vi "DE10_control.vi"() -> ()   [LabVIEW 2014]
uses:
  <vilib>/Analysis/baseanly.llb/Mean (DBL).vi
  <vilib>/Utility/file.llb/Write To Spreadsheet File (I64).vi
  <vilib>/Analysis/NI_AALBase.lvlib
panel:
  in  "Update Ch gain cal":bool
  in  "Ch Gain Cal.":T1={"A:LG"=60, "A:MG"=60, "A:HG"=60, "B:LG"=60, "B:MG"=60, "B:HG"=60, "C:LG"=60, "C:MG"=60, "C:HG"=60, "D:LG"=60, "D:MG"=60, "D:HG"=60}
  out "Average":i32=10
  in  "read back":i32=1024
  out "Counter":u16=23
  in  "Update Act ch sel":bool
  in  "Active Channel":enum32{"Ch A", "Ch B", "Ch C", "Ch D"}(radio)
  in  "flash 2 buf":bool
  in  "Write to flash":bool
  in  "Load from flash":bool
  in  "Clear Graph":bool
  out "Avg_A (uA)":dbl(graph)
  out "Peak_A (uA)":dbl(graph)
  out "Avg_A (uA)":sgl=1024.0
  in  "AFE Gain Selection":enum32{"LG", "MG", "HG"}(radio)
  in  "Register Name":u16(ring) items=["BL:G1:A", "FFIFO:WD", "BL:LEN", "EVT:TAIL", "EVT:LEN", "TRIG:DL", "TRIG:DT", "TRIG:TH", "CR", "NF:SUM", "NF:DOSX", "NF:DOSY", "THRSH", "BL:G1:A", "BL:G2:A", "BL:G3:A", "CH:SEL", "OFFS:A", "OFFS:B", "OFFS:C", "OFFS:D", "TRIP:X:MAX", "TRIP:X:MIN", "TRIP:Y:MAX", "TRIP:Y:MIN", ""]
  in  "Value (Decimal)":i32
  out "STRING OUT":string
  out "DEC  OUT":i32
  out "HEX  OUT":i32 format="%x"
  in  "Register Name 2":u16(ring) items=["", "PEAK?", "FW?", "PW?", "TRIG:DL?", "CH:SEL?", "TRIG:TH?", "BL:G3:A?", "BL:G1:C?", "BL:G2:C?", "BL:G3:C?", "BL:G1:B?", "BL:G2:B?", "BL:G3:B?", "FIFO:WD?", "FFIFO:A?", "EVT:TAIL?", "SR?", "CR?", "NF:DOS?", "NF:SUM?", "THRSH?", "X:INST?", "Y:INST?", "S:INST?", "X:AVER?", "Y:AVER?", "S:AVER?", "S:RAW?", "BL:G1:A?", "BL:G2:A?", "BL:G3:A?", "GAIN:D?", "OFFS:A?", "OFFS:B?", "OFFS:C?", "OFFS:D?", "DEBUG:A?", "DEBUG:B?", "DEBUG:C?", "DEBUG:D?", "DEBUG:MOD?", "DEBUG:BUF:A?", "DEBUG:BUF:B?", "DEBUG:BUF:C?", "DEBUG:BUF:D?", "TRIG:MASK?", "AFE:CTRL?", "TRIP:X:MAX?", "TRIP:X:MIN?", "TRIP:Y:MAX?", "TRIP:Y:MIN?", "DATA:BUF:1?", "DATA:BUF:2?", "DATA:BUF:3?", "DATA:BUF:4?", "DATA:BUF:5?"]
  in  "ARBRwrite":bool
  in  "ARBRread":bool
  out "Duty cycle (%)":sgl=1024.0
  out "Freqquency (Hz)":i32=1024
  out "pulse width(us)":i16=1024
  out "Peak_A (uA)":sgl=1024.0
  in  "FIFO clear":bool
  in  "update to flash buf":bool
  in  "MAC":i32[](array[numeric]) format="%02x"
  in  "IP":i32[](array[numeric])
  out "MB Firmware ver:":string="FPGA_VER?"
  in  "Update Ch BL":bool
  in  "Ch BL Adj.":T2={"A:BL1"=60, "A:BL2"=60, "A:BL3"=60, "B:BL1"=60, "B:BL2"=60, "B:BL3"=60, "C:BL1"=60, "C:BL2"=60, "C:BL3"=60, "DBL1"=60, "D:BL2"=60, "D:BL3"=60}
  in  "Update AFE control reg":bool
  in  "Update  mode reg":bool
  in  "Mode Register":T3={"Run"=FALSE, "External Trigger"=TRUE, "Self Trigger"=TRUE, "Internal Trigger"=TRUE, "Trigger out enable"=TRUE, "Not in use"=TRUE, "BLR readout"=TRUE, "Bypass BLR"=TRUE, "AFE Cal"=FALSE, "Not in use"=FALSE}
  in  "Update Event Parameters":bool
  in  "Event Parameters":T4={"TRIG:TH"=1000, "TRIG:DT"=0, "TRIG:DL"=300, "EVT:LEN"=1024, "EVT:TAIL"=300, "OVERSHOOT\n< 256"=100}
  out "FPGA ver:":string="FPGA_VER?"
  out "Event data path:":path
  in  "Save data":bool
  in  "Log Evt data:":bool
  out "Fast FIFO Words":i32=4096
  in  "Event Data Log":bool
  out "ADC 16 bit data RAW or after BLR/Gain Cor.":i16[](graph)
  out "AFE Conl REGISTER":bool[](array[boolean])
  out "MODE REGISTER":bool[](array[boolean])
  out "STATUS REGISTER":bool[](array[boolean])
  out "ERROR  REGISTER":bool[](array[boolean])
  out "error out":errorcluster
  in  "stop":bool
  in  "IP ADRESS":string="192.168.12.10"
  # "History:  Oct 26.2017, Jan29,2018, May29,2018,Aug21,2018\nCal: 10 uA -> 1600 @ G= 100, so I = ADC*10/(16*G)\nChannel Gain Cal: 1 ~ 511, = 1/256 ~ 511/256, so 256 is no adjust."
  # "ELinac Faraday Cup Data Acquisition/Control  Rev 1.0, SL, Oct. 26 2017"
  # "0     1     2     3     4     5     6    7      8     9    10   11   12   13    14  15"
  # "A0  A1"
  # "0     1     2     3     4     5     6    7      8     9    10   11   12   13    14  15"
  # "Run"
  # "0     1     2     3     4     5     6    7      8     9    10   11   12   13    14  15"
  # "0     1     2     3     4     5     6    7      8     9    10   11   12   13    14  15"
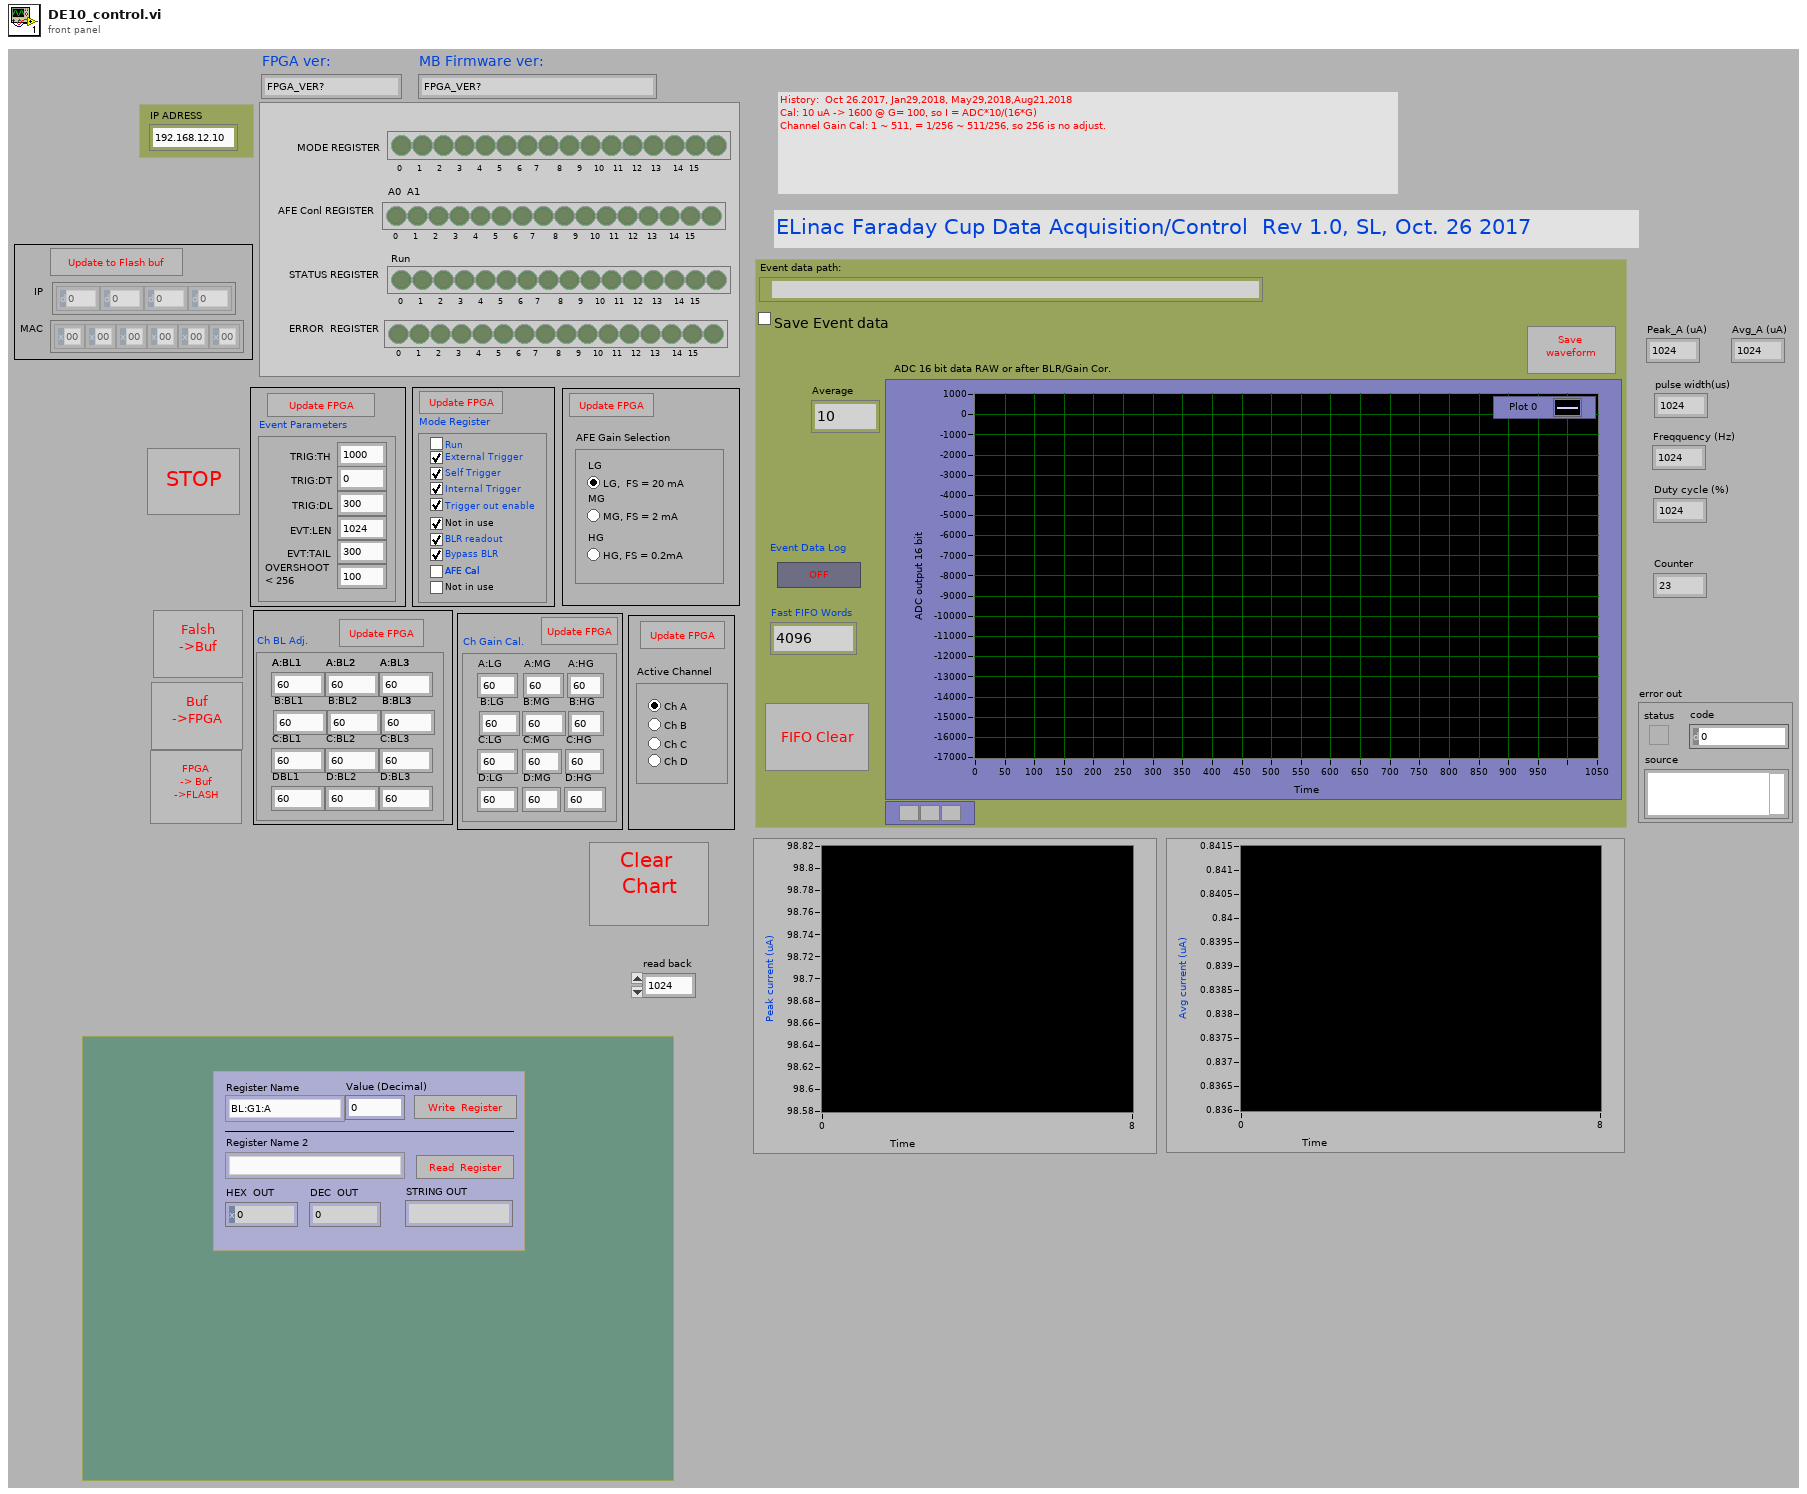
[diagram p1: front panel]
types:
  T1 = cluster{"A:LG":i16, "A:MG":i16, "A:HG":i16, "B:LG":i16, "B:MG":i16, "B:HG":i16, "C:LG":i16, "C:MG":i16, "C:HG":i16, "D:LG":i16, "D:MG":i16, "D:HG":i16}
  T2 = cluster{"A:BL1":i16, "A:BL2":i16, "A:BL3":i16, "B:BL1":i16, "B:BL2":i16, "B:BL3":i16, "C:BL1":i16, "C:BL2":i16, "C:BL3":i16, "DBL1":i16, "D:BL2":i16, "D:BL3":i16}
  T3 = cluster{"Run":bool, "External Trigger":bool, "Self Trigger":bool, "Internal Trigger":bool, "Trigger out enable":bool, "Not in use":bool, "BLR readout":bool, "Bypass BLR":bool, "AFE Cal":bool, "Not in use":bool}
  T4 = cluster{"TRIG:TH":u16, "TRIG:DT":u16, "TRIG:DL":u16, "EVT:LEN":u16, "EVT:TAIL":u16, "OVERSHOOT\n< 256":u16}
  T5 = cluster{bool, bool, bool, bool, bool, bool, bool, bool, bool, bool}
  T6 = cluster{"number out":i32, "number out":i32, "number out":i32, "number out":i32, "number out":i32, "number out":i32}
  T7 = cluster{"number out":i32, "number out":i32, "number out":i32, "number out":i32, "number out":i32, "number out":i32, "number out":i32, "number out":i32, "number out":i32, "number out":i32, "number out":i32, "number out":i32}
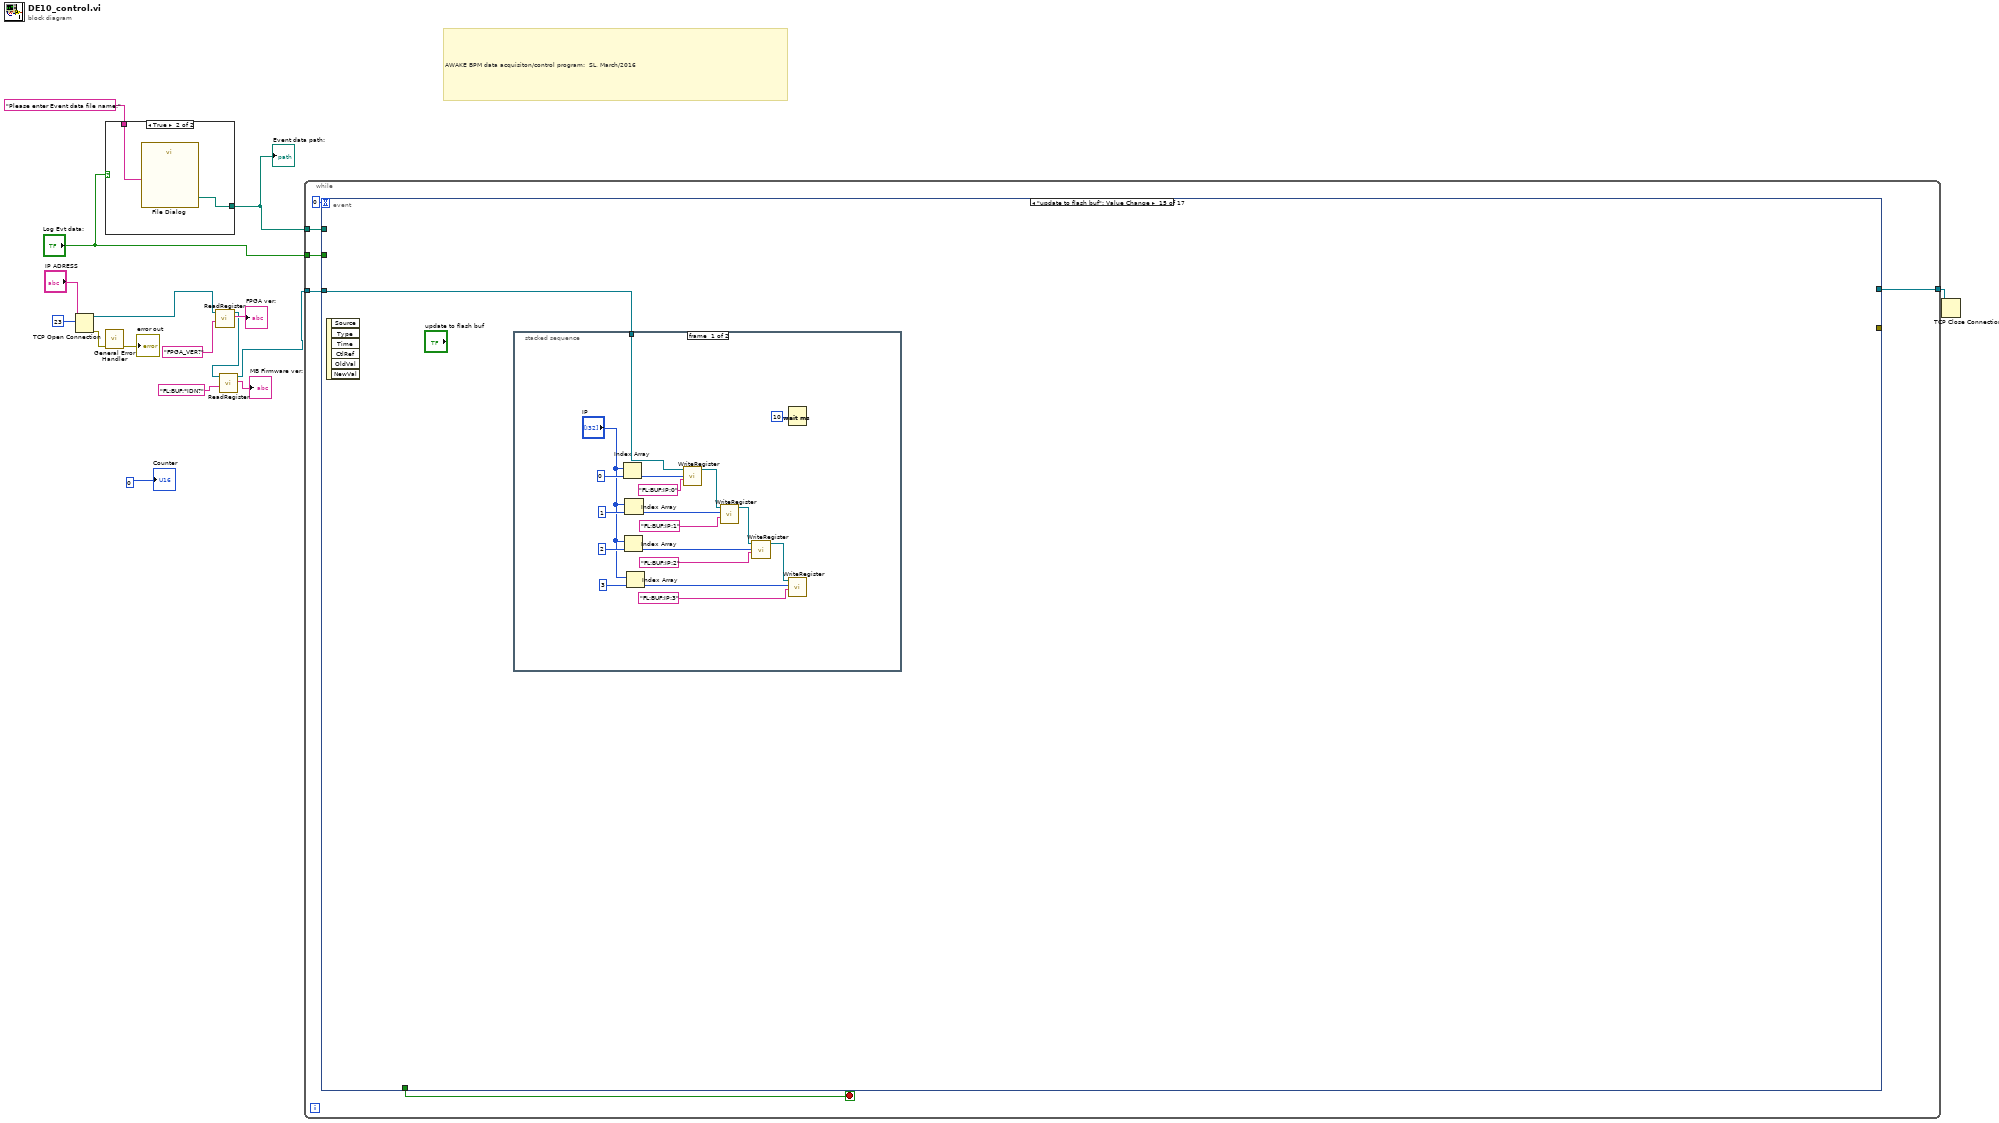
[diagram p0: block diagram]
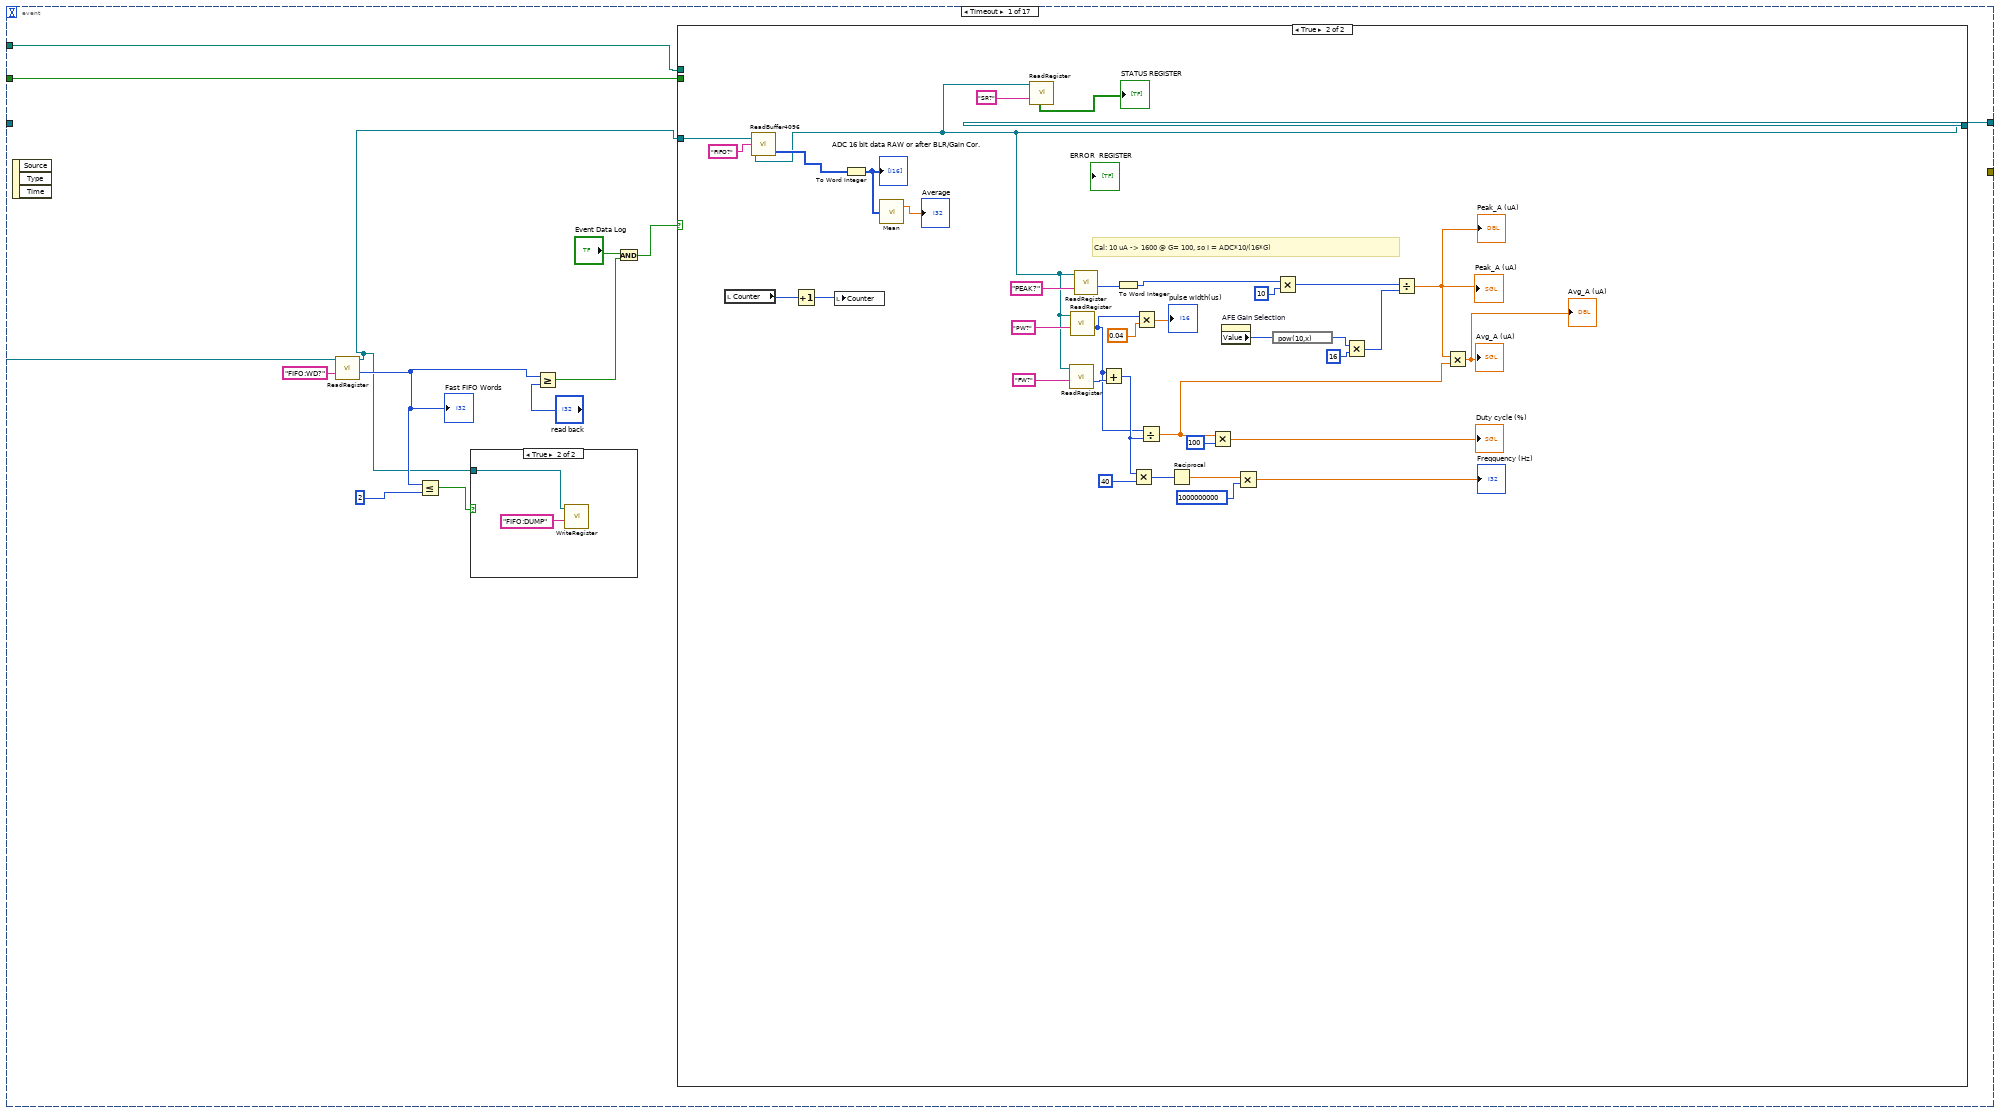
[diagram p3: hidden frame]
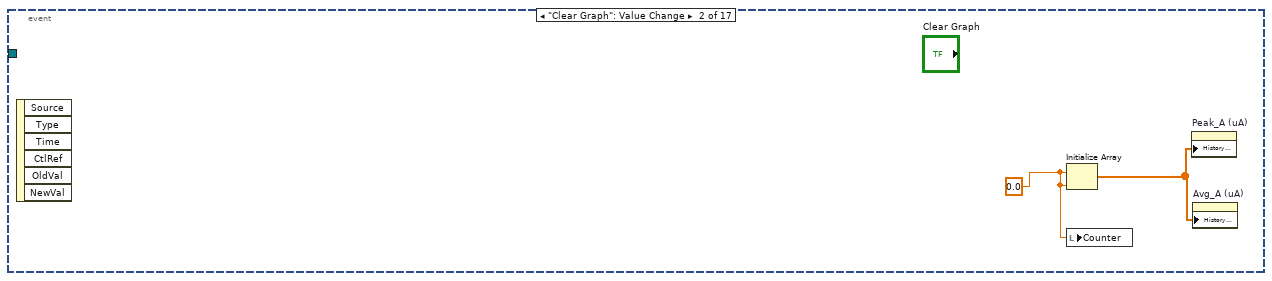
[diagram p6: hidden frame]
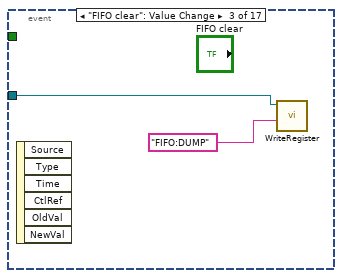
[diagram p7: hidden frame]
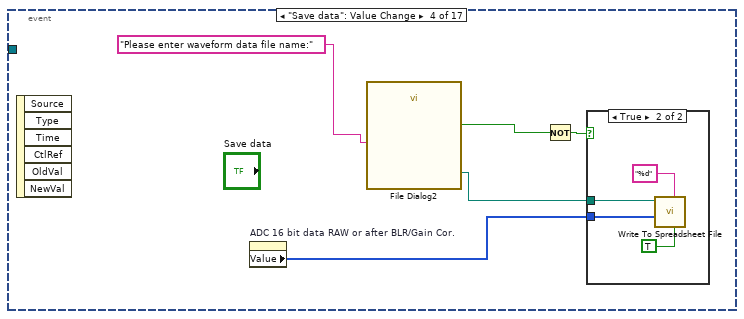
[diagram p8: hidden frame]
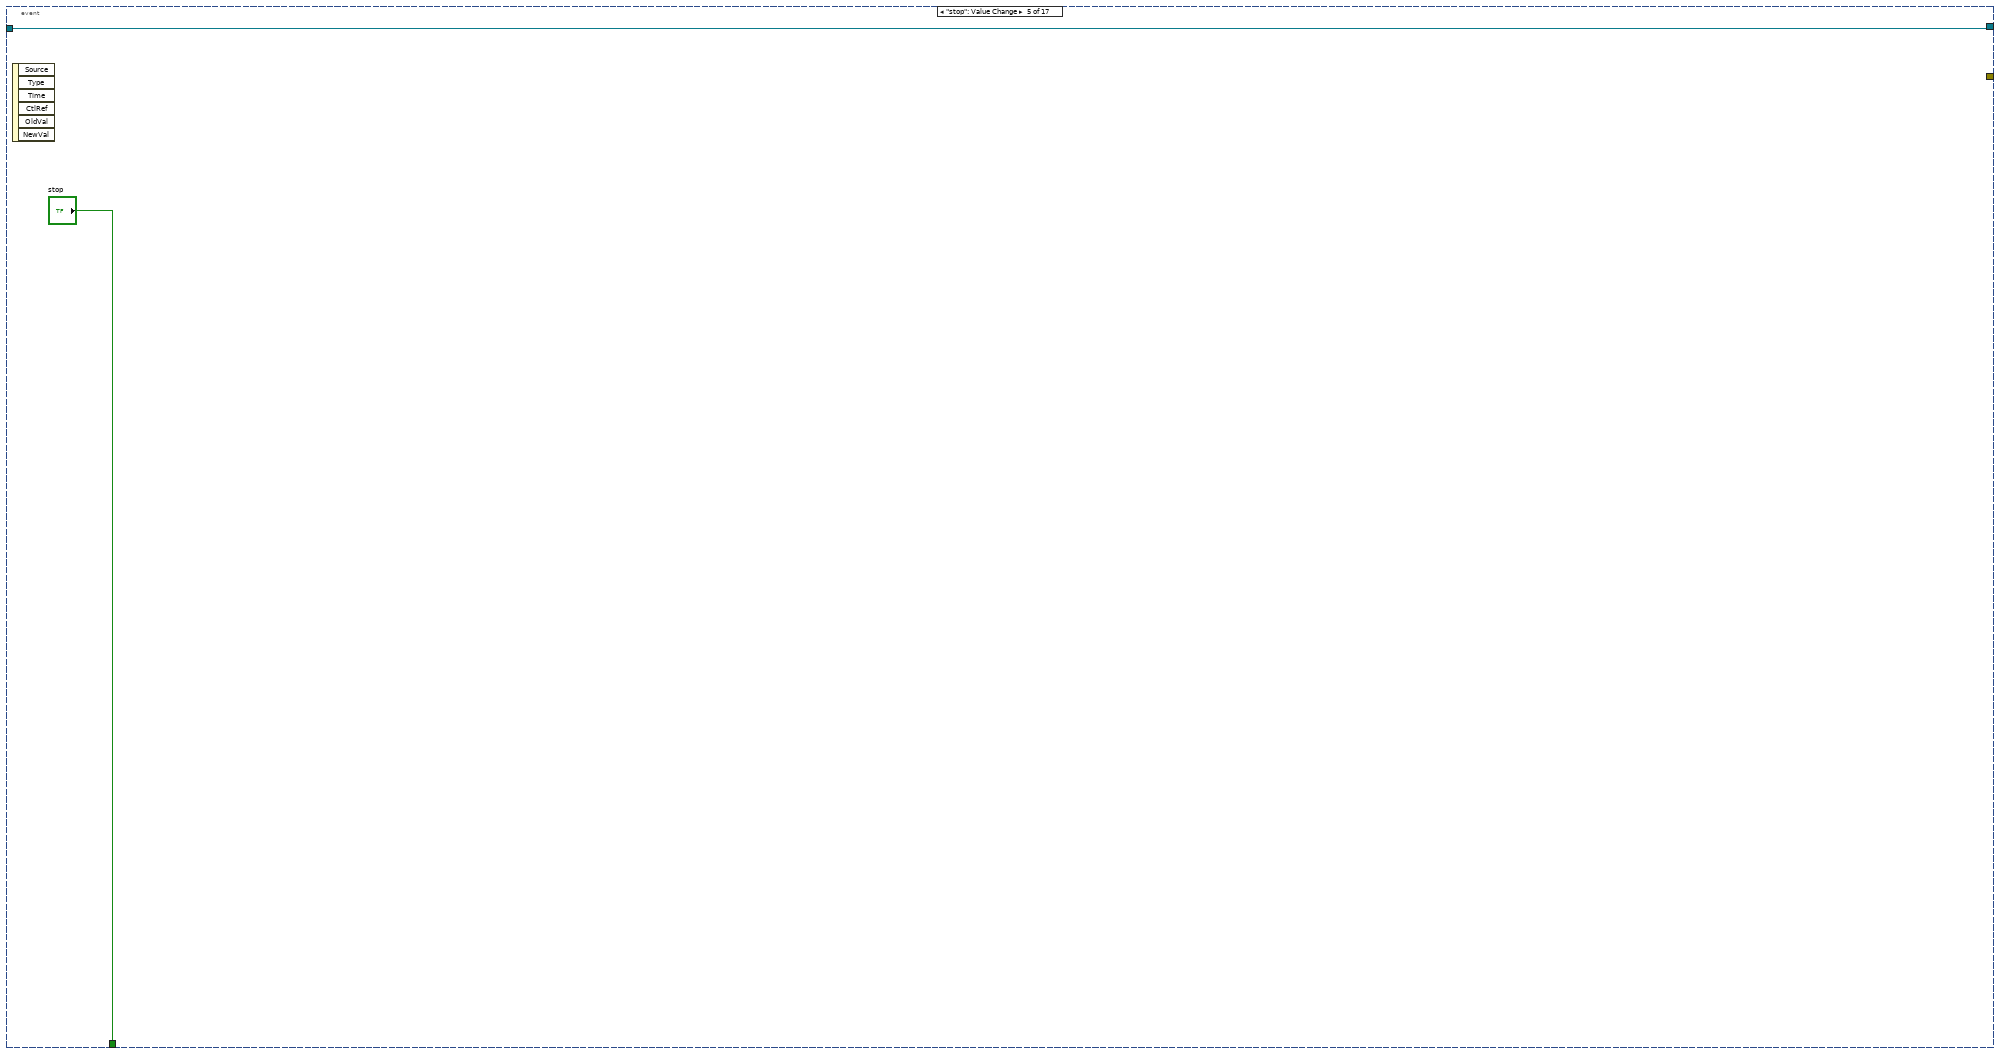
[diagram p10: hidden frame]
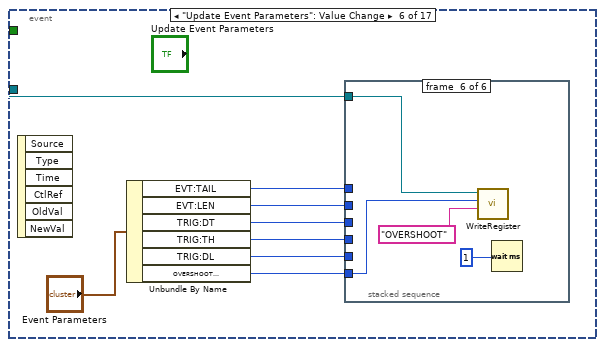
[diagram p11: hidden frame]
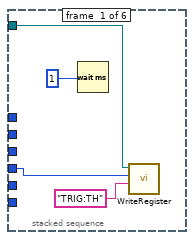
[diagram p12: hidden frame]
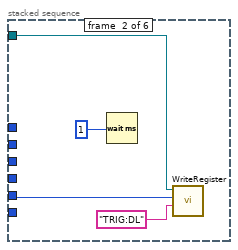
[diagram p13: hidden frame]
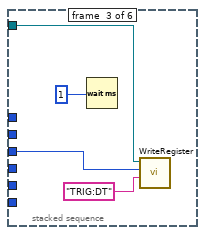
[diagram p14: hidden frame]
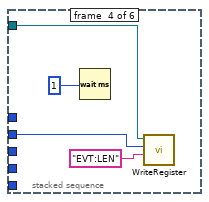
[diagram p15: hidden frame]
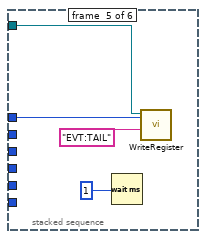
[diagram p16: hidden frame]
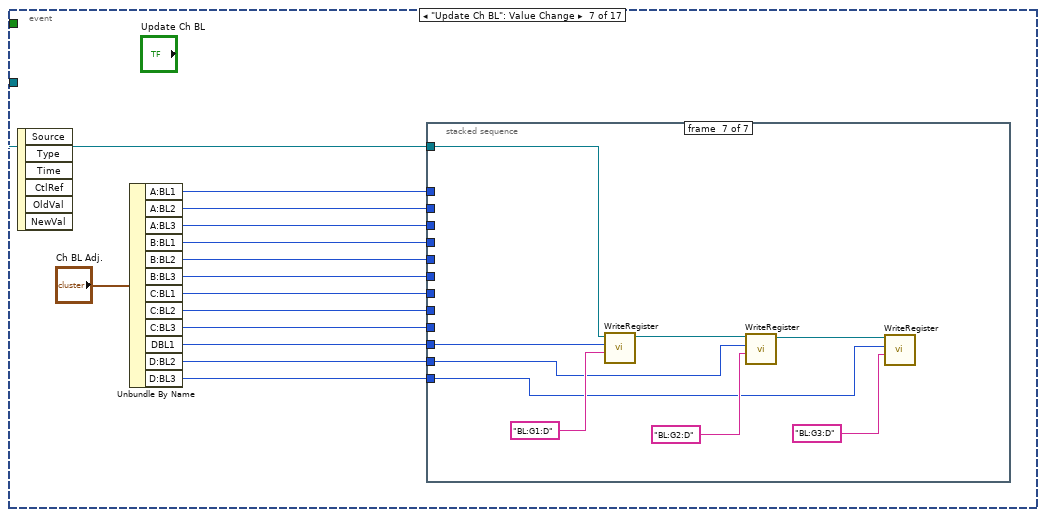
[diagram p17: hidden frame]
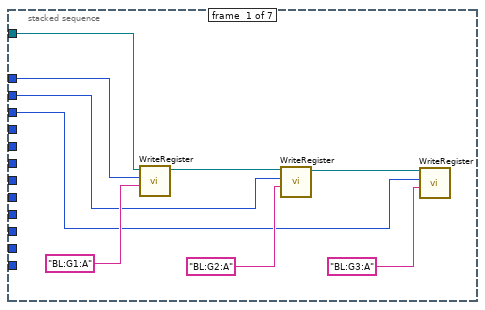
[diagram p18: hidden frame]
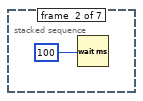
[diagram p19: hidden frame]
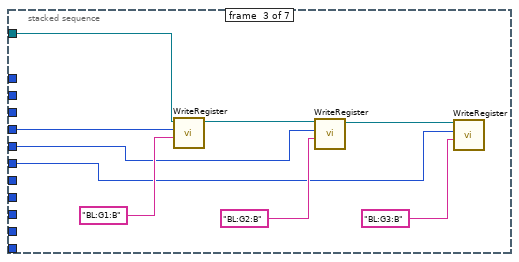
[diagram p20: hidden frame]
diagram:
  # "AWAKE BPM data acquisiton/control program:  SL, March/2016"
  n1 = TCP Open Connection(address="IP ADRESS", remote port or service name=u16 23 ("REMOTE PORT")) -> (connection ID=w8:refnum<k5>, error out=w14:errorcluster)  [unwired: 3 in]
  n2 = call <vilib>:"General Error Handler.vi"("error in (no error)"=w14) -> ("error out"=→"error out":errorcluster)  [unwired: 10 in, 4 out]
  n3 = case shown="True" "Log Evt data:" {
    tunnel: [_ w18] -> w9
    tunnel: "Please enter Event data file name:" -> [_ w17]
    frame False {
    }
    frame True {
      n4 = call "File Dialog"("prompt"=w17) -> ("selected path"=w18:path)  [unwired: 11 in, 3 out]
    }
  }
  "Event data path:" <- w9
  n5 = call "ReadRegister.vi"("string in"="FPGA_VER?", "connection ID in"=w8) -> ("string out"=→"FPGA ver:":string, "connection ID out"=w3:refnum<k5>)  [unwired: 3 in, 3 out]
  n6 = call "ReadRegister.vi"("string in"="FL:BUF:*IDN?", "connection ID in"=w3) -> ("string out"=→"MB Firmware ver:":string, "connection ID out"=w2:refnum<k5>)  [unwired: 3 in, 3 out]
  n7 = while {
    tunnel: w2 -> [w23]
    tunnel: [w22] -> w12
    tunnel: "Log Evt data:" -> [w20]
    tunnel: w9 -> [w19]
    stop <- w24 stop-if-true
    n8 = event shown="[14] \"update to flash buf\": Value Change" {
      selector: _ -> [_ _ _ _ _ _ _ _ _ _ _ _ _ _ _ _ _]
      dyn-events: _ -> [_ _ _ _ _ _ _ _ _ _ _ _ _ _ _ _ _]
      timeout: 0 -> [_ _ _ _ _ _ _ _ _ _ _ _ _ _ _ _ _]
      tunnel: [_ _ _ _ "stop" _ _ _ _ _ _ _ _ _ _ _ _] -> w24
      tunnel: w23 -> [w35 _ w79 _ w90 w94 w136 w177 w230 w233 w260 w262 w270 w416 w421 w468 w485]
      tunnel: [w36 _ _ _ w90 _ _ _ _ _ w257 _ _ _ _ _ w482] -> w22
      tunnel: [_ _ _ _ _ _ _ _ _ _ w253 _ _ _ _ _ w478] -> _
      tunnel: w20 -> [w33 _ _ _ _ _ _ _ _ _ _ _ _ _ _ _ _]
      tunnel: w19 -> [w32 _ _ _ _ _ _ _ _ _ _ _ _ _ _ _ _]
      event Timeout {
        n9 = event-data() -> ()  [unwired: 1 in, 3 out]
        n10 = call "ReadRegister.vi"("string in"="FIFO:WD?", "connection ID in"=w35) -> ("number out"=w27:i32, "connection ID out"=w25:refnum<k5>)  [unwired: 3 in, 3 out]
        "Fast FIFO Words" <- w27
        n11 = Less Or Equal?(x=w27, y=2) -> (x <= y?=w26:bool)
        n12 = case shown="True" w26 {
          tunnel: w25 -> [_ w38]
          frame False {
          }
          frame True {
            n13 = call "WriteRegister.vi"("string in"="FIFO:DUMP", "connection ID in"=w38) -> ()  [unwired: 6 in, 2 out]
          }
        }
        n14 = Greater Or Equal?(x=w27, y="read back") -> (x >= y?=w30:bool)
        n15 = And(x="Event Data Log", y=w30) -> (x .and. y?=w37:bool)
        n16 = case shown="True" w37 {
          tunnel: [w40 w46] -> w36
          tunnel: w25 -> [w40 w76]
          tunnel: w33 -> [_ _]
          tunnel: w32 -> [_ _]
          frame False {
          }
          frame True {
            # "Cal: 10 uA -> 1600 @ G= 100, so I = ADC*10/(16*G)"
            n17 = local read "Counter"() -> (w44:u16)
            n18 = call "ReadBuffer4096.vi"("string in"="FIFO?", "connection ID in"=w76) -> ("FIFO32_data"=w49:u32[], "connection ID out"=w46:refnum<k5>)  [unwired: 2 in]
            n19 = Increment(x=w44) -> (x+1=w43:u16)
            n20 = local write "Counter"(w43) -> ()
            n21 = To Word Integer(number=w49) -> (16bit integer=w42:i16[])
            "ADC 16 bit data RAW or after BLR/Gain Cor." <- w42
            n22 = call-poly <vilib>:"Mean.vi"("X"=w42) -> ("mean"=→"Average":dbl)  [unwired: 1 out]
            n23 = call "ReadRegister.vi"("string in"="SR?", "connection ID in"=w46) -> ("boolean array out"=→"STATUS REGISTER":bool[])  [unwired: 3 in, 4 out]
            n24 = call "ReadRegister.vi"("string in"="FW?", "connection ID in"=w46) -> ("number out"=w72:i32)  [unwired: 3 in, 4 out]
            n25 = call "ReadRegister.vi"("string in"="PW?", "connection ID in"=w46) -> ("number out"=w66:i32)  [unwired: 3 in, 4 out]
            n26 = call "ReadRegister.vi"("string in"="PEAK?", "connection ID in"=w46) -> ("number out"=w59:i32)  [unwired: 3 in, 4 out]
            n27 = Add(x=w66, y=w72) -> (x+y=w69:i32)
            n28 = To Word Integer(number=w59) -> (16bit integer=w58:i16)
            n29 = Multiply(x=w69, y=40) -> (x*y=w70:i32)
            n30 = Multiply(x=w66, y=0.04) -> (x*y=→"pulse width(us)":dbl)
            n31 = Divide(x=w66, y=w69) -> (x/y=w52:dbl)
            n32 = Reciprocal(x=w70) -> (1/x=w64:dbl)
            n33 = Multiply(x=w52, y=100) -> (x*y=→"Duty cycle (%)":dbl)
            n34 = property on="AFE Gain Selection" class="RadioBtnsControl (strict)"() -> ("Value"=w55:enum32{"LG", "MG", "HG"})  [unwired: 2 in, 2 out]
            n35 = Multiply(x=w64, y=1000000000) -> (x*y=→"Freqquency (Hz)":dbl)
            n36 = expression code="pow(10,x)"(w55) -> (w56:enum32{"LG", "MG", "HG"})
            n37 = Multiply(x=w58, y=10) -> (x*y=w60:i32)
            n38 = Multiply(x=w56, y=16) -> (x*y=w54:u32)
            n39 = Divide(x=w60, y=w54) -> (x/y=w51:dbl)
            "Peak_A (uA)" <- w51
            "Peak_A (uA)" <- w51
            n40 = Multiply(x=w51, y=w52) -> (x*y=→"Avg_A (uA)" →"Avg_A (uA)":dbl)
          }
        }
      }
      event "Clear Graph": Value Change {
        w77 = sgl 0.0
        n41 = event-data() -> ()  [unwired: 1 in, 6 out]
        n42 = Initialize Array(w77, w77) -> (w78:sgl[])
        n43 = local write "Counter"(w77) -> ()
        n44 = property on="Peak_A (uA)" class="WFChart (strict)"("History Data"=w78) -> ()  [unwired: 2 in, 2 out]
        n45 = property on="Avg_A (uA)" class="WFChart (strict)"("History Data"=w78) -> ()  [unwired: 2 in, 2 out]
      }
      event "FIFO clear": Value Change {
        n46 = event-data() -> ()  [unwired: 1 in, 6 out]
        n47 = call "WriteRegister.vi"("string in"="FIFO:DUMP", "connection ID in"=w79) -> ()  [unwired: 6 in, 2 out]
      }
      event "Save data": Value Change {
        n48 = event-data() -> ()  [unwired: 1 in, 6 out]
        n49 = property on="ADC 16 bit data RAW or after BLR/Gain Cor." class="WFGraph (strict)"() -> ("Value"=w82:i16[])  [unwired: 2 in, 2 out]
        n50 = call "File Dialog2"("prompt"="Please enter waveform data file name:") -> ("selected path"=w81:path, "cancelled"=w83:bool)  [unwired: 11 in, 2 out]
        n51 = Not(x=w83) -> (.not. x?=w84:bool)
        n52 = case shown="True" w84 {
          tunnel: w82 -> [_ w86]
          tunnel: w81 -> [_ w87]
          frame False {
          }
          frame True {
            n53 = call-poly <vilib>:"Write To Spreadsheet File.vi"("transpose? (no:F)"=TRUE, "format (%d)"="%d", "1D data"=w86, "file path (dialog if empty)"=w87) -> ()  [unwired: 4 in, 1 out]
          }
        }
      }
      event "stop": Value Change {
        n54 = event-data() -> ()  [unwired: 1 in, 6 out]
      }
      event "Update Event Parameters": Value Change {
        n55 = event-data() -> ()  [unwired: 1 in, 6 out]
        n56 = Unbundle By Name("Event Parameters") -> ("EVT:TAIL"=w98:u16, "EVT:LEN"=w93:u16, "TRIG:DT"=w97:u16, "TRIG:TH"=w96:u16, "TRIG:DL"=w95:u16, "OVERSHOOT\n< 256"=w92:u16)
        n57 = stacked-sequence {
          tunnel: w98 -> [_ _ _ _ w117 _]
          tunnel: w93 -> [_ _ _ w113 _ _]
          tunnel: w97 -> [_ _ w109 _ _ _]
          tunnel: w96 -> [w101 _ _ _ _ _]
          tunnel: w95 -> [_ w104 _ _ _ _]
          tunnel: w94 -> [w100 w105 w108 w112 w116 w122]
          tunnel: w92 -> [_ _ _ _ _ w121]
          frame #0 {
            n58 = Wait (ms)(milliseconds to wait=1 ("Value")) -> ()  [unwired: 1 out]
            n59 = call "WriteRegister.vi"("string in"="TRIG:TH", "value in"=w101, "connection ID in"=w100) -> ()  [unwired: 5 in, 2 out]
          }
          frame #1 {
            n60 = Wait (ms)(milliseconds to wait=1 ("Value")) -> ()  [unwired: 1 out]
            n61 = call "WriteRegister.vi"("string in"="TRIG:DL", "value in"=w104, "connection ID in"=w105) -> ()  [unwired: 5 in, 2 out]
          }
          frame #2 {
            n62 = Wait (ms)(milliseconds to wait=1 ("Value")) -> ()  [unwired: 1 out]
            n63 = call "WriteRegister.vi"("string in"="TRIG:DT", "value in"=w109, "connection ID in"=w108) -> ()  [unwired: 5 in, 2 out]
          }
          frame #3 {
            n64 = Wait (ms)(milliseconds to wait=1 ("Value")) -> ()  [unwired: 1 out]
            n65 = call "WriteRegister.vi"("string in"="EVT:LEN", "value in"=w113, "connection ID in"=w112) -> ()  [unwired: 5 in, 2 out]
          }
          frame #4 {
            n66 = Wait (ms)(milliseconds to wait=1 ("Value")) -> ()  [unwired: 1 out]
            n67 = call "WriteRegister.vi"("string in"="EVT:TAIL", "value in"=w117, "connection ID in"=w116) -> ()  [unwired: 5 in, 2 out]
          }
          frame #5 {
            n68 = call "WriteRegister.vi"("string in"="OVERSHOOT", "value in"=w121, "connection ID in"=w122) -> ()  [unwired: 5 in, 2 out]
            n69 = Wait (ms)(milliseconds to wait=1 ("Value")) -> ()  [unwired: 1 out]
          }
        }
      }
      event "Update Ch BL": Value Change {
        n70 = event-data() -> ()  [unwired: 1 in, 6 out]
        n71 = Unbundle By Name("Ch BL Adj.") -> ("A:BL1"=w135:i16, "A:BL2"=w134:i16, "A:BL3"=w133:i16, "B:BL1"=w132:i16, "B:BL2"=w131:i16, "B:BL3"=w130:i16, "C:BL1"=w129:i16, "C:BL2"=w128:i16, "C:BL3"=w127:i16, "DBL1"=w126:i16, "D:BL2"=w125:i16, "D:BL3"=w124:i16)
        n72 = stacked-sequence {
          tunnel: w136 -> [w145 _ w151 _ w161 _ w171]
          tunnel: w135 -> [w144 _ _ _ _ _ _]
          tunnel: w134 -> [w139 _ _ _ _ _ _]
          tunnel: w133 -> [w138 _ _ _ _ _ _]
          tunnel: w132 -> [_ _ w150 _ _ _ _]
          tunnel: w131 -> [_ _ w149 _ _ _ _]
          tunnel: w130 -> [_ _ w148 _ _ _ _]
          tunnel: w129 -> [_ _ _ _ w160 _ _]
          tunnel: w128 -> [_ _ _ _ w159 _ _]
          tunnel: w127 -> [_ _ _ _ w158 _ _]
          tunnel: w126 -> [_ _ _ _ _ _ w170]
          tunnel: w125 -> [_ _ _ _ _ _ w169]
          tunnel: w124 -> [_ _ _ _ _ _ w168]
          frame #0 {
            n73 = call "WriteRegister.vi"("string in"="BL:G1:A", "value in"=w144, "connection ID in"=w145) -> ("connection ID out"=w141:refnum<k5>)  [unwired: 5 in, 1 out]
            n74 = call "WriteRegister.vi"("string in"="BL:G2:A", "value in"=w139, "connection ID in"=w141) -> ("connection ID out"=w140:refnum<k5>)  [unwired: 5 in, 1 out]
            n75 = call "WriteRegister.vi"("string in"="BL:G3:A", "value in"=w138, "connection ID in"=w140) -> ()  [unwired: 5 in, 2 out]
          }
          frame #1 {
            n76 = Wait (ms)(milliseconds to wait=100 ("Value")) -> ()  [unwired: 1 out]
          }
          frame #2 {
            n77 = call "WriteRegister.vi"("string in"="BL:G1:B", "value in"=w150, "connection ID in"=w151) -> ("connection ID out"=w153:refnum<k5>)  [unwired: 5 in, 1 out]
            n78 = call "WriteRegister.vi"("string in"="BL:G2:B", "value in"=w149, "connection ID in"=w153) -> ("connection ID out"=w152:refnum<k5>)  [unwired: 5 in, 1 out]
            n79 = call "WriteRegister.vi"("string in"="BL:G3:B", "value in"=w148, "connection ID in"=w152) -> ()  [unwired: 5 in, 2 out]
          }
          frame #3 {
            n80 = Wait (ms)(milliseconds to wait=100 ("Value")) -> ()  [unwired: 1 out]
          }
          frame #4 {
            n81 = call "WriteRegister.vi"("string in"="BL:G1:C", "value in"=w160, "connection ID in"=w161) -> ("connection ID out"=w163:refnum<k5>)  [unwired: 5 in, 1 out]
            n82 = call "WriteRegister.vi"("string in"="BL:G2:C", "value in"=w159, "connection ID in"=w163) -> ("connection ID out"=w162:refnum<k5>)  [unwired: 5 in, 1 out]
            n83 = call "WriteRegister.vi"("string in"="BL:G3:C", "value in"=w158, "connection ID in"=w162) -> ()  [unwired: 5 in, 2 out]
          }
          frame #5 {
            n84 = Wait (ms)(milliseconds to wait=100 ("Value")) -> ()  [unwired: 1 out]
          }
          frame #6 {
            n85 = call "WriteRegister.vi"("string in"="BL:G1:D", "value in"=w170, "connection ID in"=w171) -> ("connection ID out"=w173:refnum<k5>)  [unwired: 5 in, 1 out]
            n86 = call "WriteRegister.vi"("string in"="BL:G2:D", "value in"=w169, "connection ID in"=w173) -> ("connection ID out"=w172:refnum<k5>)  [unwired: 5 in, 1 out]
            n87 = call "WriteRegister.vi"("string in"="BL:G3:D", "value in"=w168, "connection ID in"=w172) -> ()  [unwired: 5 in, 2 out]
          }
        }
      }
      event "Update Ch gain cal": Value Change {
        n88 = event-data() -> ()  [unwired: 1 in, 6 out]
        n89 = Unbundle By Name("Ch Gain Cal.") -> ("A:LG"=w189:i16, "A:MG"=w188:i16, "A:HG"=w187:i16, "B:LG"=w186:i16, "B:MG"=w185:i16, "B:HG"=w184:i16, "C:LG"=w183:i16, "C:MG"=w182:i16, "C:HG"=w181:i16, "D:LG"=w180:i16, "D:MG"=w179:i16, "D:HG"=w178:i16)
        n90 = stacked-sequence {
          tunnel: w177 -> [w198 _ w204 _ w214 _ w224]
          tunnel: w189 -> [w197 _ _ _ _ _ _]
          tunnel: w188 -> [w192 _ _ _ _ _ _]
          tunnel: w187 -> [w191 _ _ _ _ _ _]
          tunnel: w186 -> [_ _ w203 _ _ _ _]
          tunnel: w185 -> [_ _ w202 _ _ _ _]
          tunnel: w184 -> [_ _ w201 _ _ _ _]
          tunnel: w183 -> [_ _ _ _ w213 _ _]
          tunnel: w182 -> [_ _ _ _ w212 _ _]
          tunnel: w181 -> [_ _ _ _ w211 _ _]
          tunnel: w180 -> [_ _ _ _ _ _ w223]
          tunnel: w179 -> [_ _ _ _ _ _ w222]
          tunnel: w178 -> [_ _ _ _ _ _ w221]
          frame #0 {
            n91 = call "WriteRegister.vi"("string in"="CAL:G1:A", "value in"=w197, "connection ID in"=w198) -> ("connection ID out"=w194:refnum<k5>)  [unwired: 5 in, 1 out]
            n92 = call "WriteRegister.vi"("string in"="CAL:G2:A", "value in"=w192, "connection ID in"=w194) -> ("connection ID out"=w193:refnum<k5>)  [unwired: 5 in, 1 out]
            n93 = call "WriteRegister.vi"("string in"="CAL:G3:A", "value in"=w191, "connection ID in"=w193) -> ()  [unwired: 5 in, 2 out]
          }
          frame #1 {
            n94 = Wait (ms)(milliseconds to wait=100 ("Value")) -> ()  [unwired: 1 out]
          }
          frame #2 {
            n95 = call "WriteRegister.vi"("string in"="CAL:G1:B", "value in"=w203, "connection ID in"=w204) -> ("connection ID out"=w206:refnum<k5>)  [unwired: 5 in, 1 out]
            n96 = call "WriteRegister.vi"("string in"="CAL:G2:B", "value in"=w202, "connection ID in"=w206) -> ("connection ID out"=w205:refnum<k5>)  [unwired: 5 in, 1 out]
            n97 = call "WriteRegister.vi"("string in"="CAL:G3:B", "value in"=w201, "connection ID in"=w205) -> ()  [unwired: 5 in, 2 out]
          }
          frame #3 {
            n98 = Wait (ms)(milliseconds to wait=100 ("Value")) -> ()  [unwired: 1 out]
          }
          frame #4 {
            n99 = call "WriteRegister.vi"("string in"="CAL:G1:C", "value in"=w213, "connection ID in"=w214) -> ("connection ID out"=w216:refnum<k5>)  [unwired: 5 in, 1 out]
            n100 = call "WriteRegister.vi"("string in"="CAL:G2:C", "value in"=w212, "connection ID in"=w216) -> ("connection ID out"=w215:refnum<k5>)  [unwired: 5 in, 1 out]
            n101 = call "WriteRegister.vi"("string in"="CAL:G3:C", "value in"=w211, "connection ID in"=w215) -> ()  [unwired: 5 in, 2 out]
          }
          frame #5 {
            n102 = Wait (ms)(milliseconds to wait=100 ("Value")) -> ()  [unwired: 1 out]
          }
          frame #6 {
            n103 = call "WriteRegister.vi"("string in"="CAL:G1:D", "value in"=w223, "connection ID in"=w224) -> ("connection ID out"=w226:refnum<k5>)  [unwired: 5 in, 1 out]
            n104 = call "WriteRegister.vi"("string in"="CAL:G2:D", "value in"=w222, "connection ID in"=w226) -> ("connection ID out"=w225:refnum<k5>)  [unwired: 5 in, 1 out]
            n105 = call "WriteRegister.vi"("string in"="CAL:G3:D", "value in"=w221, "connection ID in"=w225) -> ()  [unwired: 5 in, 2 out]
          }
        }
      }
      event "ARBRwrite": Value Change {
        n106 = event-data() -> ()  [unwired: 1 in, 6 out]
        n107 = property on="Register Name" class="Ring (strict)"() -> ("RingText.Text"=w232:string)  [unwired: 2 in, 2 out]
        n108 = call "WriteRegister.vi"("string in"=w232, "value in"="Value (Decimal)", "connection ID in"=w230) -> ()  [unwired: 5 in, 2 out]
      }
      event "ARBRread": Value Change {
        n109 = event-data() -> ()  [unwired: 1 in, 6 out]
        n110 = property on="Register Name 2" class="Ring (strict)"() -> ("RingText.Text"=w236:string)  [unwired: 2 in, 2 out]
        n111 = call "ReadRegister.vi"("string in"=w236, "connection ID in"=w233) -> ("number out"=→"HEX  OUT" →"DEC  OUT":i32, "string out"=→"STRING OUT":string)  [unwired: 3 in, 3 out]
      }
      event "Update  mode reg": Value Change {
        w246 = FALSE
        n112 = event-data() -> ()  [unwired: 1 in, 6 out]
        n113 = Unbundle By Name("Mode Register") -> ("Run"=w251:bool, "Bypass BLR"=w247:bool, "BLR readout"=w248:bool, "Trigger out enable"=w239:bool, "Not in use"=w249:bool, "AFE Cal"=w250:bool, "Self Trigger"=w244:bool, "Internal Trigger"=w241:bool, "External Trigger"=w245:bool, "Not in use"=w238:bool)
        n114 = Not(x=w245) -> (.not. x?=w242:bool)
        n115 = And(x=w244, y=w242) -> (x .and. y?=w243:bool)
        n116 = And(x=w241, y=w242) -> (x .and. y?=w240:bool)
        n117 = Build Array(w251, w243, w240, w239, w239, w238, w246, w246, w248, w247, w246, w246, w246, w250, w249, w246) -> (w261:bool[])
        n118 = Boolean Array To Number(Boolean array=w261) -> (number=w237:u32)
        n119 = call "WriteRegister.vi"("string in"="CR", "value in"=w237, "connection ID in"=w260) -> ("error out"=w254:errorcluster, "connection ID out"=w258:refnum<k5>)  [unwired: 5 in]
        n120 = call "ReadRegister.vi"("error in"=w254, "string in"="CR?", "connection ID in"=w258) -> ("error out"=w253:errorcluster, "connection ID out"=w257:refnum<k5>, "boolean array out"=→"MODE REGISTER":bool[])  [unwired: 2 in, 2 out]
      }
      event "Update Act ch sel": Value Change {
        n121 = event-data() -> ()  [unwired: 1 in, 6 out]
        n122 = case shown="\"Ch A\", Default" "Active Channel" {
          tunnel: [0 1 2 3] -> w263
          frame "Ch A", Default {
          }
          frame "Ch B" {
          }
          frame "Ch C" {
          }
          frame "Ch D" {
          }
        }
        n123 = call "WriteRegister.vi"("string in"="CH:SEL", "value in"=w263, "connection ID in"=w262) -> ()  [unwired: 5 in, 2 out]
      }
      event "Load from flash": Value Change {
        n124 = event-data() -> ()  [unwired: 1 in, 6 out]
        n125 = stacked-sequence {
          tunnel: w270 -> [w271 _ w277 w295 w315 w317 w351 w395 w404]
          frame #0 {
            n126 = disable-structure shown="Enabled" {
              disable-tunnel: w271 -> [w272 _]
              frame Enabled {
                n127 = call "WriteFLBuffer.vi"("string in"="FLASHBUF:TO:FPGA", "connection ID in"=w272) -> ()  [unwired: 6 in, 2 out]
              }
              frame Disabled {
              }
            }
          }
          frame #1 {
            n128 = Wait (ms)(milliseconds to wait=200 ("Value")) -> ()  [unwired: 1 out]
          }
          frame #2 {
            n129 = call "ReadRegister.vi"("string in"="CR?", "connection ID in"=w277) -> ("boolean array out"=w276:bool[])  [unwired: 3 in, 4 out]
            n130 = local write "MODE REGISTER"(w276) -> ()
            n131 = Index Array(array=w276) -> (element #1=w280:bool, element #2=w283:bool, element #3=w286:bool, element #5=w287:bool, element #6=w288:bool, element #9=w289:bool, element #10=w290:bool, element #14=w291:bool, element #15=w292:bool)  [unwired: 16 in, 7 out]
            n132 = Not(x=w286) -> (.not. x?=w284:bool)
            n133 = Not(x=w283) -> (.not. x?=w285:bool)
            n134 = And(x=w283, y=w284) -> (x .and. y?=w281:bool)
            n135 = And(x=w285, y=w284) -> (x .and. y?=w279:bool)
            n136 = And(x=w285, y=w286) -> (x .and. y?=w282:bool)
            n137 = Bundle(w280, w279, w281, w282, w287, w288, w289, w290, w291, w292) -> (w275:T5)  [unwired: 1 in]
            n138 = local write "Mode Register"(w275) -> ()
          }
          frame #3 {
            n139 = call "ReadRegister.vi"("string in"="AFE:CTRL?", "connection ID in"=w295) -> ("number out"=w293:i32, "boolean array out"=w294:bool[])  [unwired: 3 in, 3 out]
            n140 = local write "AFE Conl REGISTER"(w294) -> ()
            n141 = property on="AFE Gain Selection" class="RadioBtnsControl (strict)"("Value"=w293) -> ()  [unwired: 2 in, 2 out]
          }
          frame #4 {
            n142 = call "ReadRegister.vi"("string in"="TRIG:TH?", "connection ID in"=w315) -> ("number out"=w305:i32, "connection ID out"=w314:refnum<k5>)  [unwired: 3 in, 3 out]
            n143 = call "ReadRegister.vi"("string in"="TRIG:DT?", "connection ID in"=w314) -> ("number out"=w304:i32, "connection ID out"=w313:refnum<k5>)  [unwired: 3 in, 3 out]
            n144 = call "ReadRegister.vi"("string in"="TRIG:DL?", "connection ID in"=w313) -> ("number out"=w303:i32, "connection ID out"=w312:refnum<k5>)  [unwired: 3 in, 3 out]
            n145 = call "ReadRegister.vi"("string in"="EVT:LEN?", "connection ID in"=w312) -> ("number out"=w302:i32, "connection ID out"=w311:refnum<k5>)  [unwired: 3 in, 3 out]
            n146 = call "ReadRegister.vi"("string in"="EVT:TAIL?", "connection ID in"=w311) -> ("number out"=w301:i32, "connection ID out"=w300:refnum<k5>)  [unwired: 3 in, 3 out]
            n147 = call "ReadRegister.vi"("string in"="OVERSHOOT?", "connection ID in"=w300) -> ("number out"=w298:i32)  [unwired: 3 in, 4 out]
            n148 = Bundle("number out"=w305, "number out"=w304, "number out"=w303, "number out"=w302, "number out"=w301, "number out"=w298) -> (w297:T6)  [unwired: 1 in]
            n149 = local write "Event Parameters"(w297) -> ()
          }
          frame #5 {
            n150 = call "ReadRegister.vi"("string in"="BL:G1:C?", "connection ID in"=w317) -> ("number out"=w328:i32, "connection ID out"=w333:refnum<k5>)  [unwired: 3 in, 3 out]
            n151 = call "ReadRegister.vi"("string in"="BL:G1:A?", "connection ID in"=w317) -> ("number out"=w344:i32, "connection ID out"=w346:refnum<k5>)  [unwired: 3 in, 3 out]
            n152 = call "ReadRegister.vi"("string in"="BL:G1:B?", "connection ID in"=w317) -> ("number out"=w331:i32, "connection ID out"=w338:refnum<k5>)  [unwired: 3 in, 3 out]
            n153 = call "ReadRegister.vi"("string in"="BL:G1:D?", "connection ID in"=w317) -> ("number out"=w320:i32, "connection ID out"=w322:refnum<k5>)  [unwired: 3 in, 3 out]
            n154 = call "ReadRegister.vi"("string in"="BL:G2:C?", "connection ID in"=w333) -> ("number out"=w327:i32, "connection ID out"=w332:refnum<k5>)  [unwired: 3 in, 3 out]
            n155 = call "ReadRegister.vi"("string in"="BL:G2:A?", "connection ID in"=w346) -> ("number out"=w343:i32, "connection ID out"=w345:refnum<k5>)  [unwired: 3 in, 3 out]
            n156 = call "ReadRegister.vi"("string in"="BL:G2:B?", "connection ID in"=w338) -> ("number out"=w330:i32, "connection ID out"=w337:refnum<k5>)  [unwired: 3 in, 3 out]
            n157 = call "ReadRegister.vi"("string in"="BL:G2:D?", "connection ID in"=w322) -> ("number out"=w319:i32, "connection ID out"=w321:refnum<k5>)  [unwired: 3 in, 3 out]
            n158 = call "ReadRegister.vi"("string in"="BL:G3:C?", "connection ID in"=w332) -> ("number out"=w326:i32)  [unwired: 3 in, 4 out]
            n159 = call "ReadRegister.vi"("string in"="BL:G3:A?", "connection ID in"=w345) -> ("number out"=w342:i32)  [unwired: 3 in, 4 out]
            n160 = call "ReadRegister.vi"("string in"="BL:G3:B?", "connection ID in"=w337) -> ("number out"=w329:i32)  [unwired: 3 in, 4 out]
            n161 = call "ReadRegister.vi"("string in"="BL:G3:D?", "connection ID in"=w321) -> ("number out"=w318:i32)  [unwired: 3 in, 4 out]
            n162 = Bundle "Bundle"("number out"=w344, "number out"=w343, "number out"=w342, "number out"=w331, "number out"=w330, "number out"=w329, "number out"=w328, "number out"=w327, "number out"=w326, "number out"=w320, "number out"=w319, "number out"=w318) -> (w316:T7)  [unwired: 1 in]
            n163 = local write "Ch BL Adj."(w316) -> ()
          }
          frame #6 {
            n164 = call "ReadRegister.vi"("string in"="CAL:G1:C?", "connection ID in"=w351) -> ("number out"=w362:i32, "connection ID out"=w367:refnum<k5>)  [unwired: 3 in, 3 out]
            n165 = call "ReadRegister.vi"("string in"="CAL:G1:A?", "connection ID in"=w351) -> ("number out"=w378:i32, "connection ID out"=w380:refnum<k5>)  [unwired: 3 in, 3 out]
            n166 = call "ReadRegister.vi"("string in"="CAL:G1:B?", "connection ID in"=w351) -> ("number out"=w365:i32, "connection ID out"=w372:refnum<k5>)  [unwired: 3 in, 3 out]
            n167 = call "ReadRegister.vi"("string in"="CAL:G1:D?", "connection ID in"=w351) -> ("number out"=w354:i32, "connection ID out"=w356:refnum<k5>)  [unwired: 3 in, 3 out]
            n168 = call "ReadRegister.vi"("string in"="CAL:G2:C?", "connection ID in"=w367) -> ("number out"=w361:i32, "connection ID out"=w366:refnum<k5>)  [unwired: 3 in, 3 out]
            n169 = call "ReadRegister.vi"("string in"="CAL:G2:A?", "connection ID in"=w380) -> ("number out"=w377:i32, "connection ID out"=w379:refnum<k5>)  [unwired: 3 in, 3 out]
            n170 = call "ReadRegister.vi"("string in"="CAL:G2:B?", "connection ID in"=w372) -> ("number out"=w364:i32, "connection ID out"=w371:refnum<k5>)  [unwired: 3 in, 3 out]
            n171 = call "ReadRegister.vi"("string in"="CAL:G2:D?", "connection ID in"=w356) -> ("number out"=w353:i32, "connection ID out"=w355:refnum<k5>)  [unwired: 3 in, 3 out]
            n172 = call "ReadRegister.vi"("string in"="CAL:G3:C?", "connection ID in"=w366) -> ("number out"=w360:i32)  [unwired: 3 in, 4 out]
            n173 = call "ReadRegister.vi"("string in"="CAL:G3:A?", "connection ID in"=w379) -> ("number out"=w376:i32)  [unwired: 3 in, 4 out]
            n174 = call "ReadRegister.vi"("string in"="CAL:G3:B?", "connection ID in"=w371) -> ("number out"=w363:i32)  [unwired: 3 in, 4 out]
            n175 = call "ReadRegister.vi"("string in"="CAL:G3:D?", "connection ID in"=w355) -> ("number out"=w352:i32)  [unwired: 3 in, 4 out]
            n176 = Bundle "Bundle"("number out"=w378, "number out"=w377, "number out"=w376, "number out"=w365, "number out"=w364, "number out"=w363, "number out"=w362, "number out"=w361, "number out"=w360, "number out"=w354, "number out"=w353, "number out"=w352) -> (w350:T7)  [unwired: 1 in]
            n177 = local write "Ch Gain Cal."(w350) -> ()
          }
          frame #7 {
            n178 = call "ReadRegister.vi"("string in"="FL:BUF:IP:0?", "connection ID in"=w395) -> ("number out"=w388:i32, "connection ID out"=w391:refnum<k5>)  [unwired: 3 in, 3 out]
            n179 = call "ReadRegister.vi"("string in"="FL:BUF:IP:1?", "connection ID in"=w391) -> ("number out"=w387:i32, "connection ID out"=w390:refnum<k5>)  [unwired: 3 in, 3 out]
            n180 = call "ReadRegister.vi"("string in"="FL:BUF:IP:2?", "connection ID in"=w390) -> ("number out"=w386:i32, "connection ID out"=w389:refnum<k5>)  [unwired: 3 in, 3 out]
            n181 = call "ReadRegister.vi"("string in"="FL:BUF:IP:3?", "connection ID in"=w389) -> ("number out"=w385:i32)  [unwired: 3 in, 4 out]
            n182 = Build Array(w388, w387, w386, w385) -> (w384:i32[])
            n183 = local write "IP"(w384) -> ()
          }
          frame #8 {
            n184 = call "ReadRegister.vi"("string in"="FL:BUF:MAC:0?", "connection ID in"=w404) -> ("number out"=w408:i32, "connection ID out"=w411:refnum<k5>)  [unwired: 3 in, 3 out]
            n185 = call "ReadRegister.vi"("string in"="FL:BUF:MAC:1?", "connection ID in"=w411) -> ("number out"=w407:i32, "connection ID out"=w410:refnum<k5>)  [unwired: 3 in, 3 out]
            n186 = call "ReadRegister.vi"("string in"="FL:BUF:MAC:2?", "connection ID in"=w410) -> ("number out"=w406:i32, "connection ID out"=w409:refnum<k5>)  [unwired: 3 in, 3 out]
            n187 = call "ReadRegister.vi"("string in"="FL:BUF:MAC:3?", "connection ID in"=w409) -> ("number out"=w405:i32, "connection ID out"=w401:refnum<k5>)  [unwired: 3 in, 3 out]
            n188 = call "ReadRegister.vi"("string in"="FL:BUF:MAC:4?", "connection ID in"=w401) -> ("number out"=w399:i32, "connection ID out"=w400:refnum<k5>)  [unwired: 3 in, 3 out]
            n189 = call "ReadRegister.vi"("string in"="FL:BUF:MAC:5?", "connection ID in"=w400) -> ("number out"=w398:i32)  [unwired: 3 in, 4 out]
            n190 = Build Array(w408, w407, w406, w405, w399, w398) -> (w397:i32[])
            n191 = local write "MAC"(w397) -> ()
          }
        }
      }
      event "flash 2 buf": Value Change {
        n192 = event-data() -> ()  [unwired: 1 in, 6 out]
        n193 = Two Button Dialog(message="Load parameters from FLASH to Labview? ") -> (T button?=w417:bool)  [unwired: 2 in]
        n194 = case shown="True" w417 {
          tunnel: w416 -> [_ w419]
          frame False {
          }
          frame True {
            n195 = call "WriteFLBuffer.vi"("string in"="FLASH:READ", "connection ID in"=w419) -> ()  [unwired: 6 in, 2 out]
          }
        }
      }
      event "update to flash buf": Value Change {
        n196 = event-data() -> ()  [unwired: 1 in, 6 out]
        n197 = stacked-sequence {
          tunnel: w421 -> [w423 w441]
          frame #0 {
            n198 = Index Array(array="IP", index=0) -> (element=w435:i32)
            n199 = Index Array(array="IP", index=2) -> (element=w426:i32)
            n200 = Index Array(array="IP", index=1) -> (element=w424:i32)
            n201 = Index Array(array="IP", index=3) -> (element=w428:i32)
            n202 = call "WriteRegister.vi"("string in"="FL:BUF:IP:0", "value in"=w435, "connection ID in"=w423) -> ("connection ID out"=w430:refnum<k5>)  [unwired: 5 in, 1 out]
            n203 = call "WriteRegister.vi"("string in"="FL:BUF:IP:1", "value in"=w424, "connection ID in"=w430) -> ("connection ID out"=w431:refnum<k5>)  [unwired: 5 in, 1 out]
            n204 = call "WriteRegister.vi"("string in"="FL:BUF:IP:2", "value in"=w426, "connection ID in"=w431) -> ("connection ID out"=w432:refnum<k5>)  [unwired: 5 in, 1 out]
            n205 = Wait (ms)(milliseconds to wait=u32 10) -> ()  [unwired: 1 out]
            n206 = call "WriteRegister.vi"("string in"="FL:BUF:IP:3", "value in"=w428, "connection ID in"=w432) -> ()  [unwired: 5 in, 2 out]
          }
          frame #1 {
            n207 = Index Array(array="MAC", index=0) -> (element=w449:i32)
            n208 = Index Array(array="MAC", index=2) -> (element=w463:i32)
            n209 = Index Array(array="MAC", index=1) -> (element=w465:i32)
            n210 = Index Array(array="MAC", index=3) -> (element=w461:i32)
            n211 = Index Array(array="MAC", index=4) -> (element=w456:i32)
            n212 = Index Array(array="MAC", index=5) -> (element=w454:i32)
            n213 = call "WriteRegister.vi"("string in"="FL:BUF:MAC:0", "value in"=w449, "connection ID in"=w441) -> ("connection ID out"=w459:refnum<k5>)  [unwired: 5 in, 1 out]
            n214 = call "WriteRegister.vi"("string in"="FL:BUF:MAC:1", "value in"=w465, "connection ID in"=w459) -> ("connection ID out"=w458:refnum<k5>)  [unwired: 5 in, 1 out]
            n215 = call "WriteRegister.vi"("string in"="FL:BUF:MAC:2", "value in"=w463, "connection ID in"=w458) -> ("connection ID out"=w457:refnum<k5>)  [unwired: 5 in, 1 out]
            n216 = call "WriteRegister.vi"("string in"="FL:BUF:MAC:3", "value in"=w461, "connection ID in"=w457) -> ("connection ID out"=w452:refnum<k5>)  [unwired: 5 in, 1 out]
            n217 = call "WriteRegister.vi"("string in"="FL:BUF:MAC:4", "value in"=w456, "connection ID in"=w452) -> ("connection ID out"=w451:refnum<k5>)  [unwired: 5 in, 1 out]
            n218 = Wait (ms)(milliseconds to wait=u32 10) -> ()  [unwired: 1 out]
            n219 = call "WriteRegister.vi"("string in"="FL:BUF:MAC:5", "value in"=w454, "connection ID in"=w451) -> ()  [unwired: 5 in, 2 out]
          }
        }
      }
      event "Write to flash": Value Change {
        n220 = event-data() -> ()  [unwired: 1 in, 6 out]
        n221 = Two Button Dialog(message="FPGA parameters will be written to FLASH buffer and FLASH!") -> (T button?=w466:bool)  [unwired: 2 in]
        n222 = case shown="True" w466 {
          tunnel: w468 -> [_ w469]
          frame False {
          }
          frame True {
            n223 = stacked-sequence {
              tunnel: w469 -> [w471 w474]
              frame #0 {
                n224 = Wait (ms)(milliseconds to wait=200 ("Value")) -> ()  [unwired: 1 out]
                n225 = call "WriteFLBuffer.vi"("string in"="FPGA:TO:FLASHBUF", "connection ID in"=w471) -> ()  [unwired: 6 in, 2 out]
              }
              frame #1 {
                n226 = Wait (ms)(milliseconds to wait=200 ("Value")) -> ()  [unwired: 1 out]
                n227 = call "WriteFLBuffer.vi"("string in"="FLASH:WRIT", "connection ID in"=w474) -> ()  [unwired: 6 in, 2 out]
              }
            }
          }
        }
      }
      event "Update AFE control reg": Value Change {
        n228 = event-data() -> ()  [unwired: 1 in, 6 out]
        n229 = case shown="\"MG\"" "AFE Gain Selection" {
          tunnel: [1 2 3] -> w476
          frame "LG", Default {
          }
          frame "MG" {
          }
          frame "HG" {
          }
        }
        n230 = call "WriteRegister.vi"("string in"="AFE:CTRL", "value in"=w476, "connection ID in"=w485) -> ("error out"=w479:errorcluster, "connection ID out"=w483:refnum<k5>)  [unwired: 5 in]
        n231 = call "ReadRegister.vi"("error in"=w479, "string in"="AFE:CTRL?", "connection ID in"=w483) -> ("error out"=w478:errorcluster, "connection ID out"=w482:refnum<k5>, "boolean array out"=→"AFE Conl REGISTER":bool[])  [unwired: 2 in, 2 out]
      }
    }
  }
  n232 = TCP Close Connection(connection ID=w12) -> ()  [unwired: 2 in, 2 out]
  "Counter" <- u16 0 ("REMOTE PORT")
